vi "Get Array References.vi"(8 "error in (no error)":errorcluster, 10 "Name":string, 11 "json class in":refnum<class "json class.lvclass">) -> (0 "error out":errorcluster, 2 "Array json class":refnum<class "json class.lvclass">[](array[class]), 3 "json class out":refnum<class "json class.lvclass">)   [LabVIEW 2021, in "Config Library.lvlib" / "json class.lvclass"]
uses:
  json class.lvclass
  json class.lvclass/json class.ctl
  <vilib>/addons/JSON API/JSON Value/JSON Value.lvclass
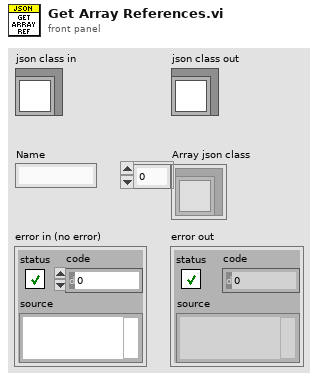
[diagram p1: front panel]
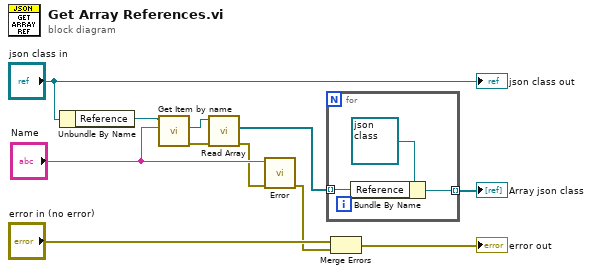
[diagram p0: block diagram]
diagram:
  n1 = Unbundle By Name("json class in") -> ("Reference"=w6:refnum<class "JSON Value.lvclass">)
  n2 = call-dynamic "Get Item by name.vi"("name"="Name", "JSON Value In"=w6) -> ("error out"=w4:errorcluster, "Value"=w5:refnum<class "JSON Value.lvclass">)  [unwired: 6 in, 2 out]
  n3 = call-dynamic "Read Array.vi"("error in (no error)"=w4, "JSON Value In"=w5) -> ("error out"=w2:errorcluster, "Array"=w7:refnum<class "JSON Value.lvclass">[])  [unwired: 7 in, 1 out]
  n4 = call "Error.vi"("error in (no error)"=w2, "Name"="Name") -> ("error out"=w1:errorcluster)  [unwired: 9 in]
  n5 = for {
    tunnel: w7 -> [w14] mode=indexing
    tunnel: [w12] -> w9 mode=indexing
    n6 = Bundle By Name(cluster=refnum<class "json class.lvclass"> refnum ("json class in"), "Reference"=w14) -> (w12:refnum<class "json class.lvclass">)
  }
  "Array json class" <- w9
  n7 = Merge Errors("error in (no error)", w1) -> (→"error out":errorcluster)
  "json class out" <- "json class in"
